vi "CalcExpress - Close Instance.vi"(6 "error in":bool, 9 "CE InstanceRef":T1) -> (0 "error out":bool, 1 "destroyed":bool, 3 "dup CE InstanceRef":T1)   [LabVIEW 2021]
doc: "The VI destroys a dynamic CalcExpress instance context or reinitializes static one.\n\nThis basic (low-level) VI has boolean error connectors instead of traditional error clusters. For more convenience, you can use top-level CalcExpress VIs that use error clusters.\n\nFor more information, see help for this VI.\n\n::: CalcExpress Toolkit :::\nCopyright (c) 2000-2026 Konstantin Shifershteyn. All rights reserved."
uses:
  cetypes.llb/CalcExpress Instance RefNum.ctl
  cersrc/celveng32.dll
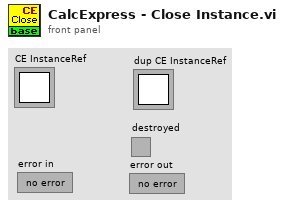
[diagram p1: front panel]
types:
  T1 = typedef "CalcExpress Instance RefNum.ctl" = refnum<k1>
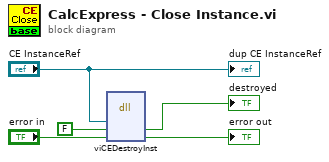
[diagram p0: block diagram]
diagram:
  n1 = dll-call lib="C:/LV Projects/CalcExpress 40 LV2021/vi.lib/addons/CalcExpress/cersrc/celveng*.dll" fn="viCEDestroyInst"("iRef"="CE InstanceRef", "fDestroyed"=FALSE, "erf"="error in") -> ("fDestroyed"=→"destroyed":bool, "erf"=→"error out":bool)  [unwired: 5 in, 2 out]
  "dup CE InstanceRef" <- "CE InstanceRef"
